vi "Initialize Result.vi"(8 "error in (no error)":errorcluster, 11 "SQL Statement":refnum<class "SQL Statement.lvclass">) -> (0 "error out":errorcluster, 3 "PGJDPResult out":refnum<class "Result.lvclass">)   [LabVIEW 2020, in "ORM_sqlite_jdp.lvlib" / "Result.lvclass"]
uses:
  Result.lvclass
  <vilib>/drjdpowell/SQLite Library/SQL Statement/SQL Statement.lvclass
  Result.lvclass/Result.ctl
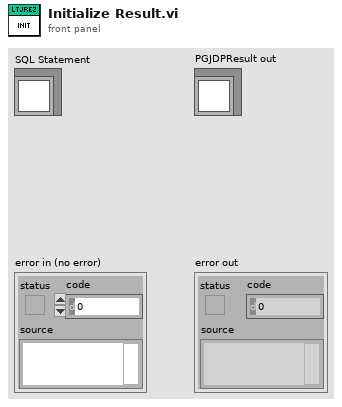
[diagram p1: front panel]
types:
  T1 = cluster{"SQL Statement":refnum<class "SQL Statement.lvclass">, "Headers":string[], "DeclaredTypes":string[]}
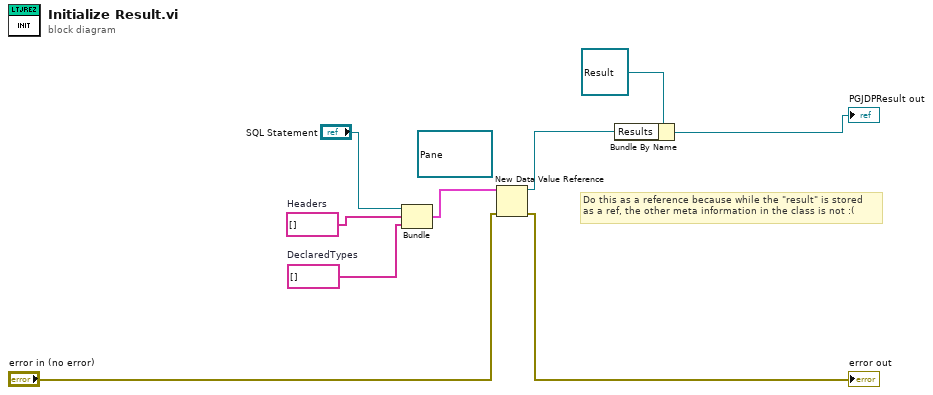
[diagram p0: block diagram]
diagram:
  (unwired) refnum<data-value> refnum ("data value reference")
  w3 = string[] []  # DeclaredTypes
  w4 = string[] []  # Headers
  # "Do this as a reference because while the \"result\" is stored\nas a ref, the other meta information in the class is not :("
  n1 = Bundle("SQL Statement"="SQL Statement", "Headers"=w4, "DeclaredTypes"=w3) -> (w2:T1)  [unwired: 1 in]
  n2 = New Data Value Reference(data value=w2, error in="error in (no error)") -> (data value reference=w1:refnum<data-value>, error out=→"error out":errorcluster)
  n3 = Bundle By Name(cluster=refnum<class "Result.lvclass"> refnum ("PGJDPResult out"), "Results"=w1) -> (→"PGJDPResult out":refnum<class "Result.lvclass">)
